vi "Cleanup.vi"(8 "error in (no error)":errorcluster, 11 "Node in":refnum<class "bt_Composite.lvclass">) -> (0 "error out":errorcluster, 3 "Node out":refnum<class "bt_Composite.lvclass">)   [LabVIEW 2021, in "BT.lvlib" / "bt_Composite.lvclass"]
uses:
  bt_Composite.lvclass
  bt_Composite.lvclass/bt_Composite.ctl
  abs_Node/bt_Node.lvclass
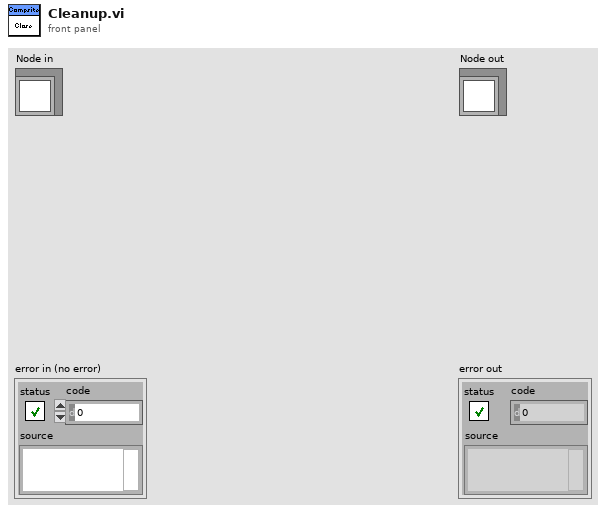
[diagram p1: front panel]
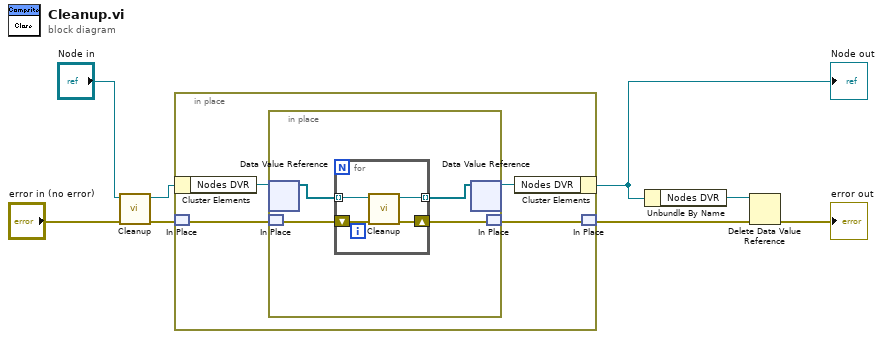
[diagram p0: block diagram]
diagram:
  n1 = call-parent "Cleanup.vi"("error in (no error)"="error in (no error)", "Node in"="Node in") -> ("error out"=w4:errorcluster, "Node out"=w3:refnum<class "bt_Composite.lvclass">)  [unwired: 8 in]
  n2 = in-place {
    n3 = in-place-cluster #1(w3) -> ("Nodes DVR"=w12:refnum<data-value>)
    n4 = in-place-match #2(w4) -> (w10:errorcluster)
    n5 = in-place {
      n6 = in-place-dvr #3(w12) -> (w14:refnum<class "bt_Node.lvclass">[])  [unwired: 1 out]
      n7 = in-place-match #4(w10) -> (w16:errorcluster)
      n8 = for {
        tunnel: w14 -> [w18] mode=indexing
        tunnel: [w17] -> w13 mode=indexing
        shift-right: [w19] -> w15
        shift-left: w16 -> [w20]
        n9 = call-dynamic "Cleanup.vi"("error in (no error)"=w20, "Node in"=w18) -> ("error out"=w19:errorcluster, "Node out"=w17:refnum<class "bt_Node.lvclass">)  [unwired: 8 in]
      }
      n10 = in-place-dvr #3(w13) -> (w11:refnum<data-value>)  [unwired: 1 out]
      n11 = in-place-match #4(w15) -> (w9:errorcluster)
    }
    n12 = in-place-cluster #1("Nodes DVR"=w11) -> (w2:refnum<class "bt_Composite.lvclass">)
    n13 = in-place-match #2(w9) -> (w1:errorcluster)
  }
  "Node out" <- w2
  n14 = Unbundle By Name(w2) -> ("Nodes DVR"=w6:refnum<data-value>)
  n15 = Delete Data Value Reference(data value reference=w6, error in=w1) -> (error out=→"error out":errorcluster)  [unwired: 1 out]
